vi "VIH Project - Get New & Supposed Old Menu Item Paths.vi"(8 "error in":errorcluster, 9 "Test File Type (T)":bool=TRUE, 10 "old Menu Path":path, 11 "new Menu Path":path) -> (0 "error out":errorcluster, 2 "Supposed Old Item Paths":path[](array[path]), 3 "New Item Paths":path[](array[path]))   [LabVIEW 2014]
doc: "::: VI Helpeks :::\nCopyright (c) 2000-2026 Konstantin Shifershteyn. All rights reserved."
uses:
  _VIH HelpGen - Palette.llb/VIH HelpGen Typedef - Palette - Item Type Enum.ctl
panel:
  # "VI Helpeks\nCopyright (c) 2012-2026 Konstantin Shifershteyn"
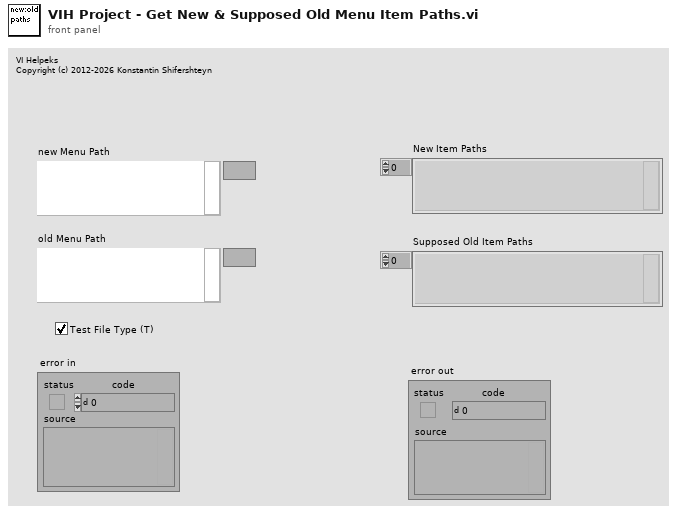
[diagram p1: front panel]
types:
  T1 = typedef "VIH HelpGen Typedef - Palette - Item Type Enum.ctl" = enum32{"<Invalid>", "<unknown>", "VI", "Menu", "LV Func", "Express VI", "Poly VI", "CTL", "HTML"}
  T2 = typedef "VIH HelpGen Typedef - Palette - Item Info Cluster.ctl" = cluster{"Item Type":T1, "Item Name":string, "Item File":path, "Parent palette":path, "Not found":bool}
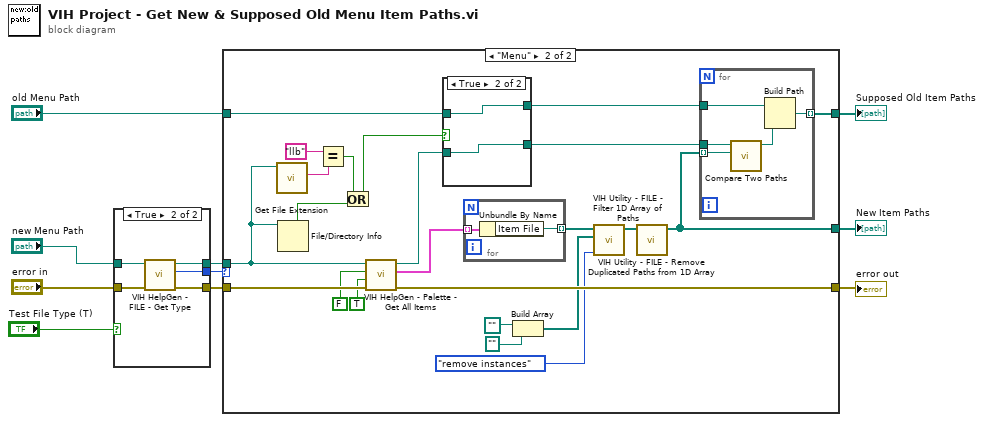
[diagram p0: block diagram]
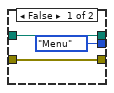
[diagram p2: hidden frame]
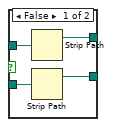
[diagram p4: hidden frame]
diagram:
  n1 = case shown="True" "Test File Type (T)" {
    tunnel: [VIH_HelpGen_Typedef_-_Palette_-_Item_Type_Enum."Menu" ("File Type") w18] -> w10
    tunnel: [w13 w17] -> w9
    tunnel: [w12 w16] -> w7
    tunnel: "new Menu Path" -> [w13 w15]
    tunnel: "error in" -> [w12 w14]
    frame False {
    }
    frame True {
      n2 = call "VIH HelpGen - FILE - Get Type.vi"("error in"=w14, "File Path"=w15) -> ("error out"=w16:errorcluster, "File Type"=w18:T1, "dup File Path"=w17:path)  [unwired: 7 in]
    }
  }
  n3 = case shown="\"Menu\"" w10 {
    tunnel: w9 -> [_ w25]
    tunnel: "old Menu Path" -> [_ w42]
    tunnel: w7 -> [w19 w40]
    tunnel: [w19 w41] -> w6
    tunnel: [_ w27] -> w3
    tunnel: [_ w26] -> w2
    frame Default {
    }
    frame "Menu" {
      n4 = call <vilib>:"Get File Extension.vi"("file"=w25) -> ("lowercase file extension"=w24:string)  [unwired: 7 in, 3 out]
      n5 = File/Directory Info(path=w25) -> (directory=w21:bool)  [unwired: 1 in, 6 out]
      n6 = Equal?(x="llb", y=w24) -> (x = y?=w22:bool)
      n7 = Or(x=w22, y=w21) -> (x .or. y?=w20:bool)
      n8 = call "VIH HelpGen - Palette - Get All Items.vi"("error in"=w40, "Entire hierarchy (T)"=TRUE, "Include master menu (T)"=FALSE, "Palette Path"=w25) -> ("error out"=w41:errorcluster, "Items Array"=w35:T2[], "dup Palette Path"=w38:path)  [unwired: 5 in]
      n9 = case shown="True" w20 {
        tunnel: w42 -> [w46 w48]
        tunnel: w38 -> [w45 w47]
        tunnel: [w44 w47] -> w37
        tunnel: [w43 w48] -> w36
        frame False {
          n10 = Strip Path(path=w46) -> (stripped path=w43:path)  [unwired: 1 out]
          n11 = Strip Path(path=w45) -> (stripped path=w44:path)  [unwired: 1 out]
        }
        frame True {
        }
      }
      n12 = for {
        tunnel: w35 -> [w50] mode=indexing
        tunnel: [w49] -> w34 mode=indexing
        n13 = Unbundle By Name(w50) -> ("Item File"=w49:path)
      }
      n14 = Build Array(path "", path "") -> (w31:path[])
      n15 = call "VIH Utility - FILE - Filter 1D Array of Paths.vi"("Action (keep instances)"=enum16{"keep instances", "remove instances"}."remove instances", "Instances"=w31, "Paths in"=w34) -> ("Paths out"=w29:path[])  [unwired: 4 in]
      n16 = call "VIH Utility - FILE - Remove Duplicated Paths from 1D Array.vi"("Array in"=w29) -> ("Array out"=w27:path[])  [unwired: 9 in, 1 out]
      n17 = for {
        tunnel: w37 -> [w55]
        tunnel: w36 -> [w54]
        tunnel: w27 -> [w52] mode=indexing
        tunnel: [w51] -> w26 mode=indexing
        n18 = call <vilib>:"Compare Two Paths.vi"("Path 2"=w52, "Path 1"=w55) -> ("Relative Path from 1 to 2"=w53:path)  [unwired: 6 in, 3 out]
        n19 = Build Path(base path=w54, name or relative path=w53) -> (appended path=w51:path)
      }
    }
  }
  "error out" <- w6
  "New Item Paths" <- w3
  "Supposed Old Item Paths" <- w2
